vi "HP8903 Get Input sample rate.vi"(0 "VISA session":refnum<visa-resource-name>, 3 "error in (no error)":errorcluster) -> (6 "dup VISA session":refnum<visa-resource-name>, 7 "SamplingRate":string, 10 "error out":errorcluster)   [LabVIEW 8.6]
doc: "This vi configures the frequency, amplitude, frequency and amplitude increment values, and the ouput impedance of the audio analyzer's source."
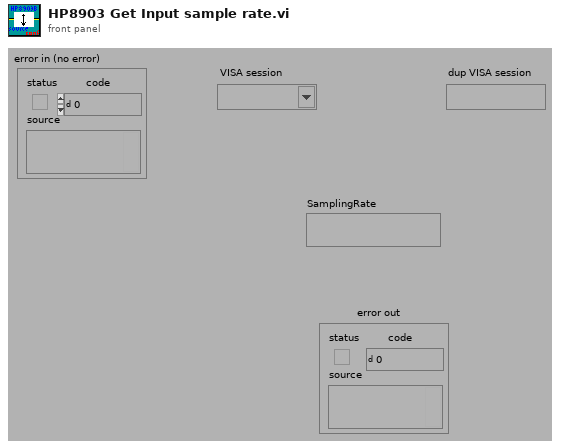
[diagram p1: front panel]
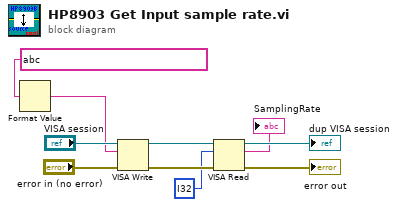
[diagram p0: block diagram]
diagram:
  n1 = Format Value(format string=string ?) -> (output string=w7:string)  [unwired: 2 in]
  n2 = VISA Write(VISA resource name="VISA session", write buffer=w7, error in (no error)="error in (no error)") -> (VISA resource name out=w6:refnum<visa-resource-name>, error out=w5:errorcluster)  [unwired: 1 out]
  n3 = VISA Read(VISA resource name=w6, byte count=i32 ?, error in (no error)=w5) -> (VISA resource name out=→"dup VISA session":refnum<visa-resource-name>, read buffer=→"SamplingRate":string, error out=→"error out":errorcluster)  [unwired: 1 out]
